vi "SUP_Camera_Queue_Latest.vi"(11 "packet":variant) -> (0 "telemetry error":errorcluster caption="sortie d'erreur", 3 "replaced_or_error":bool)   [LabVIEW 2012]
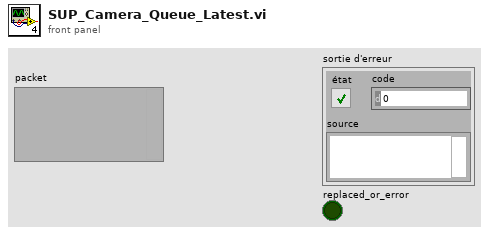
[diagram p1: front panel]
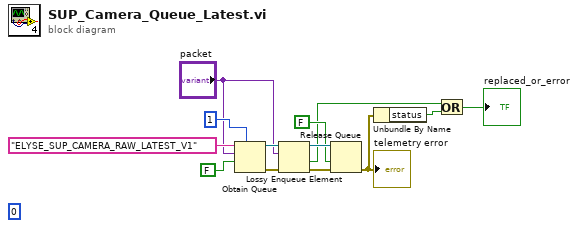
[diagram p0: block diagram]
diagram:
  (unwired) 0 ("timeout en ms (-1)")
  n1 = Obtain Queue(max queue size (-1, unlimited)=1 ("taille max de la file d'attente (-1, non limitée)"), name (unnamed)="ELYSE_SUP_CAMERA_RAW_LATEST_V1" ("nom (aucun)"), element data type="packet", create if not found? (T)=FALSE ("créer si introuvable ? (V)")) -> (queue out=w10:refnum<queue>, error out=w1:errorcluster)  [unwired: 1 in, 1 out]
  n2 = Lossy Enqueue Element(queue=w10, element="packet", error in (no error)=w1) -> (queue out=w8:refnum<queue>, overflow?=w3:bool, error out=w7:errorcluster)  [unwired: 1 out]
  n3 = Release Queue(queue=w8, force destroy? (F)=FALSE ("forcer la destruction ? (F)"), error in (no error)=w7) -> (error out=w5:errorcluster)  [unwired: 2 out]
  "telemetry error" <- w5
  n4 = Unbundle By Name(w5) -> ("status"=w4:bool)
  n5 = Or(x=w3, y=w4) -> (x .or. y?=→"replaced_or_error":bool)
